vi "Low-Level Write.vi"(5 "Finished? (True)":bool=TRUE, 6 "Mask payload?":bool, 7 "Opcode (Text)":T1=1 items=["Cont. Frame"=0, "Text"=1, "Binary"=2, "Ping"=9, "Pong"=10], 8 "error in (no error)":errorcluster, 9 "timeout ms (5000)":i32=5000, 10 "Data":u8[](array[numeric]), 11 "WebSockets in":refnum<class "WebSocket.lvclass">) -> (0 "error out":errorcluster, 3 "WebSockets out":refnum<class "WebSocket.lvclass">)   [LabVIEW 2013, in "WebSockets.lvlib" / "WebSocket.lvclass"]
doc: "Sends a WebSocket frame to the connection endpoint. Messages sent from the client must be masked but it is optional for the server.\n\nFinished should be set to True unless sending a fragmented message."
uses:
  WebSocket.lvclass
  Opcodes.ctl
panel:
  # "(leave as 'True' unless sending fragmented messages)"
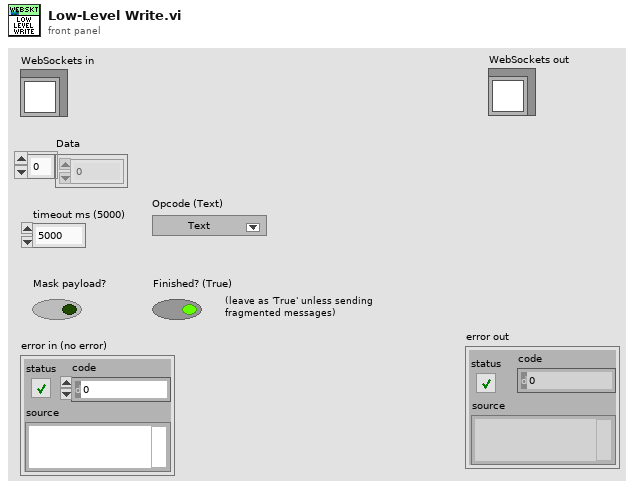
[diagram p1: front panel]
types:
  T1 = typedef "WebSockets.lvlib/WebSocket.lvclass/Opcodes.ctl" = u8
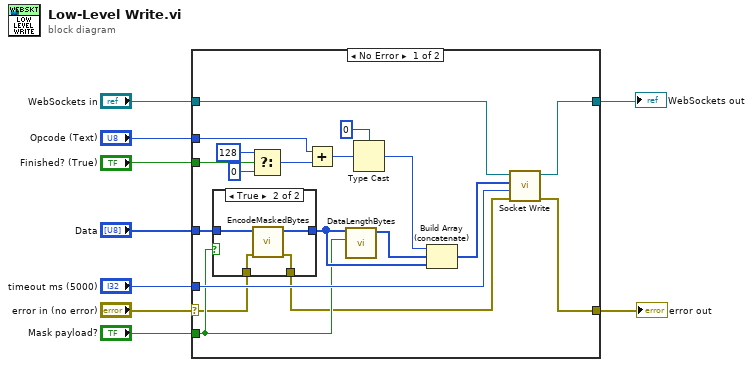
[diagram p0: block diagram]
diagram:
  n1 = case shown="No Error" "error in (no error)" {
    selector: "error in (no error)" -> [w20 w36]
    tunnel: [w28 w36] -> w8
    tunnel: [w10 w35] -> w2
    tunnel: "WebSockets in" -> [w11 w35]
    tunnel: "Data" -> [w23 _]
    tunnel: "timeout ms (5000)" -> [w24 _]
    tunnel: "Mask payload?" -> [w21 _]
    tunnel: "Finished? (True)" -> [w18 _]
    tunnel: "Opcode (Text)" -> [w16 _]
    frame No Error {
      n2 = case shown="True" w21 {
        tunnel: w23 -> [w30 w34]
        tunnel: [w30 w33] -> w22
        tunnel: w20 -> [w29 w32]
        tunnel: [w29 w31] -> w19
        frame False {
        }
        frame True {
          n3 = call "EncodeMaskedBytes.vi"("error in (no error)"=w32, "Raw Data"=w34) -> ("error out"=w31:errorcluster, "Masked Data"=w33:u8[])  [unwired: 8 in]
        }
      }
      n4 = Select(t=u8 128, s=w18, f=u8 0) -> (s? t:f=w17:u8)
      n5 = Add(x=w16, y=w17) -> (x+y=w26:T1)
      n6 = call "DataLengthBytes.vi"("Is masked?"=w21, "Data"=w22) -> ("Length Bytes"=w27:u8[])  [unwired: 9 in]
      n7 = Type Cast(type=u8 0 ("f"), x=w26) -> (*(type *) &x=w13:u8)
      n8 = Build Array (concatenate)(w13, w27, w22) -> (w25:u8[])
      n9 = call "Socket Write.vi"("error in (no error)"=w19, "timeout ms (5000)"=w24, "Bytes to write"=w25, "WebSocket in"=w11) -> ("error out"=w28:errorcluster, "WebSocket out"=w10:refnum<class "WebSocket.lvclass">)  [unwired: 5 in, 1 out]
    }
    frame Error {
    }
  }
  "error out" <- w8
  "WebSockets out" <- w2
